vi "W01_Packer_test.vi"() -> ()   [LabVIEW 2026]
doc: "Use this template to build a VI to use as a subVI."
panel:
  out "reject[]":bool[](array[boolean])
  out "grade[]":string[](array[string])
  out "why[]":string[](array[string])
  out "run[]":bool[](array[boolean])
  out "all[]":bool[](array[boolean])
  in  "weight[]":dbl[](array[numeric])
  in  "stop[]":bool[](array[boolean])
  in  "start[]":bool[](array[boolean])
  in  "Auto mode []":bool[](array[boolean])
  in  "Downstream ready []":bool[](array[boolean])
  in  "Film loaded []":bool[](array[boolean])
  in  "Seal temperature reached []":bool[](array[boolean])
  in  "Air pressure OK []":bool[](array[boolean])
  in  "E-stop released []":bool[](array[boolean])
  in  "Door 2 closed []":bool[](array[boolean])
  in  "Door 1 closed []":bool[](array[boolean])
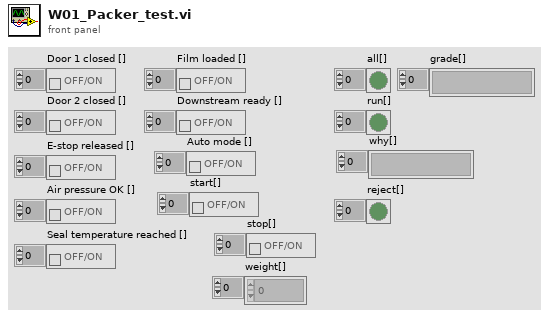
[diagram p1: front panel]
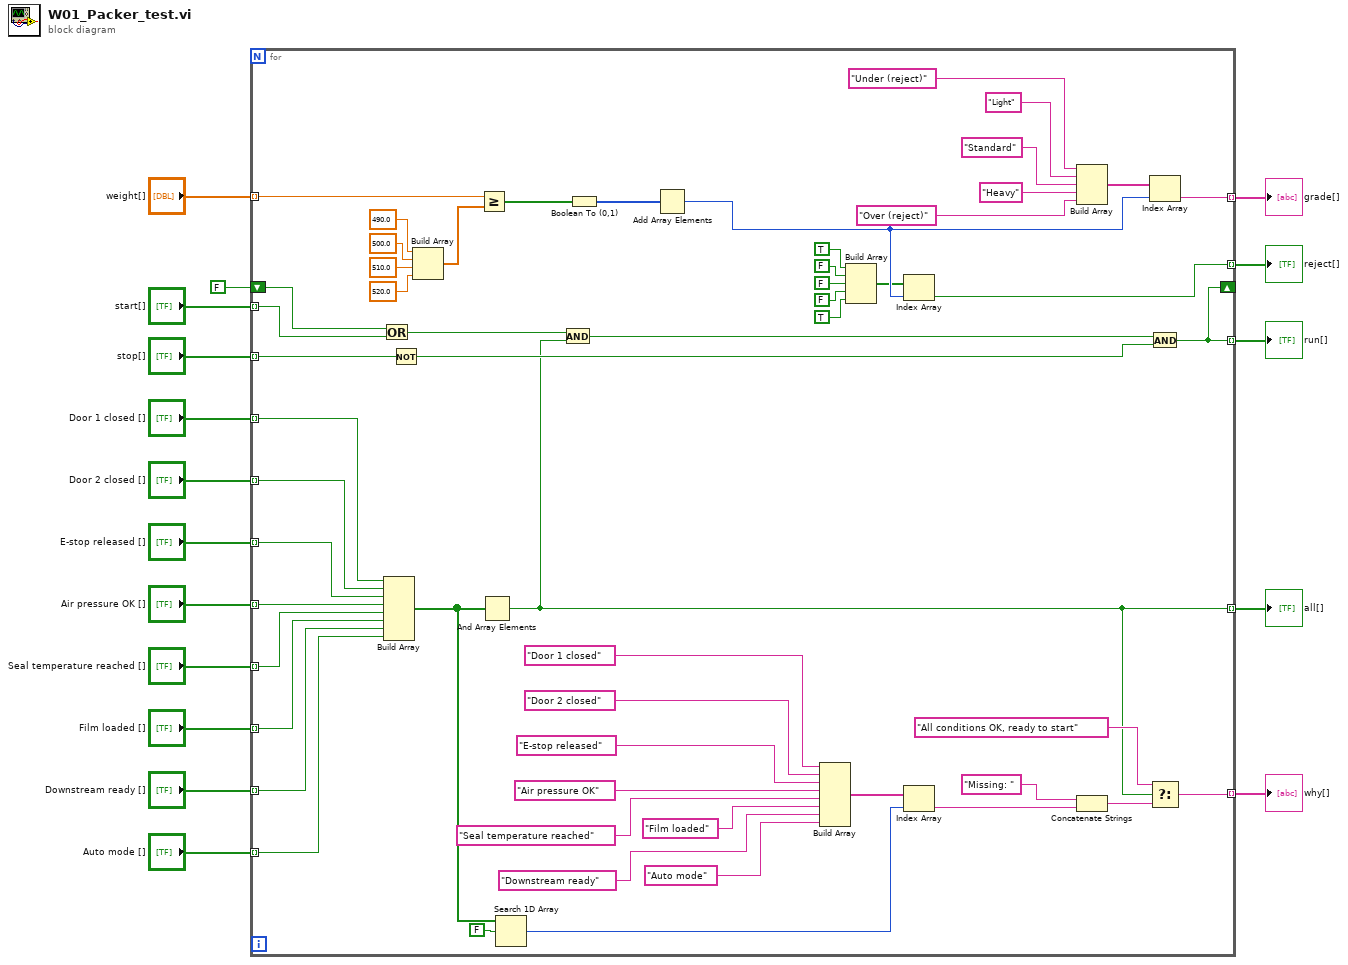
[diagram p0: block diagram]
diagram:
  n1 = for {
    shift-right: [w21] -> _
    shift-left: FALSE -> [w49]
    tunnel: "Door 1 closed []" -> [w73] mode=indexing
    tunnel: "Door 2 closed []" -> [w72] mode=indexing
    tunnel: "E-stop released []" -> [w71] mode=indexing
    tunnel: "Air pressure OK []" -> [w70] mode=indexing
    tunnel: "Seal temperature reached []" -> [w69] mode=indexing
    tunnel: "Film loaded []" -> [w68] mode=indexing
    tunnel: "Downstream ready []" -> [w67] mode=indexing
    tunnel: "Auto mode []" -> [w66] mode=indexing
    tunnel: "start[]" -> [w48] mode=indexing
    tunnel: "stop[]" -> [w46] mode=indexing
    tunnel: "weight[]" -> [w43] mode=indexing
    tunnel: [w22] -> w5 mode=indexing
    tunnel: [w21] -> w4 mode=indexing
    tunnel: [w20] -> w3 mode=indexing
    tunnel: [w19] -> w2 mode=indexing
    tunnel: [w18] -> w1 mode=indexing
    n2 = Or(x=w49, y=w48) -> (x .or. y?=w47:bool)
    n3 = Build Array(w73, w72, w71, w70, w69, w68, w67, w66) -> (w65:bool[])
    n4 = Not(x=w46) -> (.not. x?=w44:bool)
    n5 = Build Array(490.0 ("x"), 500.0 ("x"), 510.0 ("x"), 520.0 ("x")) -> (w38:dbl[])
    n6 = Greater Or Equal?(x=w43, y=w38) -> (x >= y?=w37:bool[])
    n7 = And Array Elements(Boolean array=w65) -> (logical AND=w22:bool)
    n8 = Search 1D Array(1D array=w65, element=FALSE) -> (index of element=w54:i32)  [unwired: 1 in]
    n9 = And(x=w47, y=w22) -> (x .and. y?=w45:bool)
    n10 = Boolean To (0,1)(Boolean=w37) -> (0, 1=w36:i16[])
    n11 = Add Array Elements(numeric array=w36) -> (sum=w29:i16)
    n12 = Build Array("Door 1 closed", "Door 2 closed", "E-stop released", "Air pressure OK", "Seal temperature reached", "Film loaded", "Downstream ready", "Auto mode") -> (w55:string[])
    n13 = Build Array(TRUE, FALSE, FALSE, FALSE, TRUE) -> (w23:bool[])
    n14 = Index Array(array=w23, index=w29) -> (element=w18:bool)
    n15 = Index Array(array=w55, index=w54) -> (element=w52:string)
    n16 = Build Array("Under (reject)", "Light", "Standard", "Heavy", "Over (reject)") -> (w30:string[])
    n17 = Concatenate Strings("Missing: ", w52) -> (w50:string)
    n18 = Index Array(array=w30, index=w29) -> (element=w19:string)
    n19 = And(x=w45, y=w44) -> (x .and. y?=w21:bool)
    n20 = Select(t="All conditions OK, ready to start", s=w22, f=w50) -> (s? t:f=w20:string)
  }
  "all[]" <- w5
  "run[]" <- w4
  "why[]" <- w3
  "grade[]" <- w2
  "reject[]" <- w1
